vi "LB_FocusName_Tests.vi"(11 "error in":errorcluster) -> (15 "error out":errorcluster)   [LabVIEW 2016, in "DronaTest.lvlib"]
uses:
  DronaTest.lvlib
  APIs/Stimulus/ControlValue/SetValueAuto.vi
  APIs/Stimulus/ControlValue/Controls/Listbox/SetValueByItemName.vi
  APIs/Assert/AssertControlValue/Controls/Listbox/AssertValueByFocusName.vi
  APIs/Assert/AssertControlValue/Controls/Listbox/AssertValueByFocusIndex.vi
  <vilib>/addons/_JKI Toolkits/Caraya/classes/Assert/Assert Error.vi
  <vilib>/addons/_JKI Toolkits/Caraya/classes/Assert/Assert Equal Value_Variant.vi
  <vilib>/addons/_JKI Toolkits/Caraya/classes/Test/Test.lvclass
  Drona.lvlib
  <vilib>/SLL Toolkit/SLL Debug/SLL Debug.lvlib
  APIs/Stimulus/ControlValue/ControlValue.lvlib
  <vilib>/addons/_JKI Toolkits/Caraya/classes/Assert/Assert.lvclass
  APIs/Assert/AssertControlValue/Controls/Listbox/AssertListbox.lvlib
  APIs/Stimulus/ControlValue/Controls/Listbox/StimulusListbox.lvlib
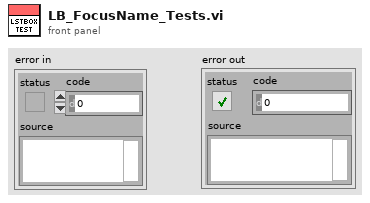
[diagram p1: front panel]
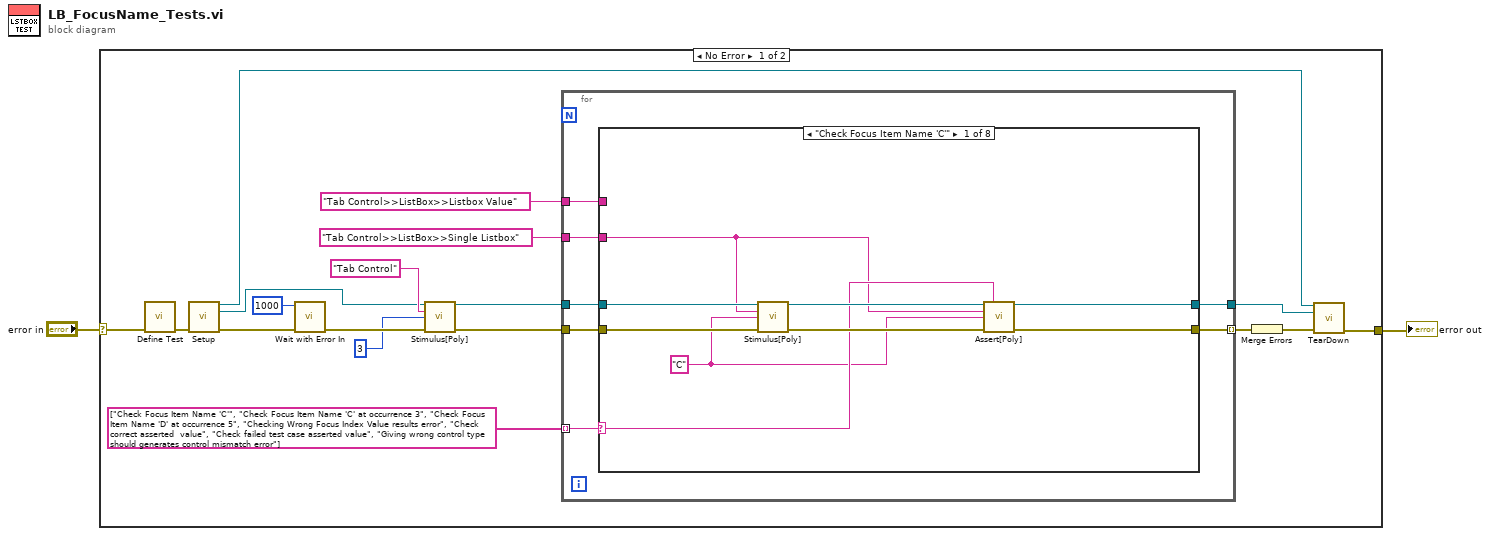
[diagram p0: block diagram]
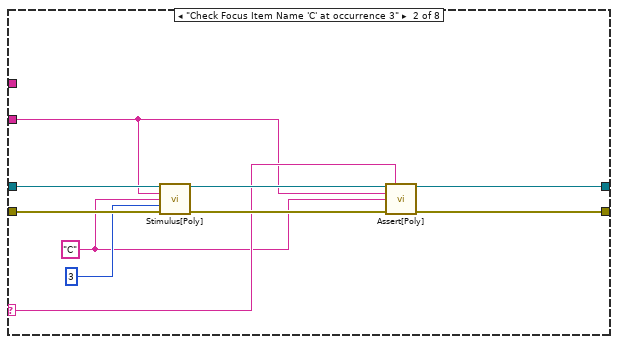
[diagram p2: hidden frame]
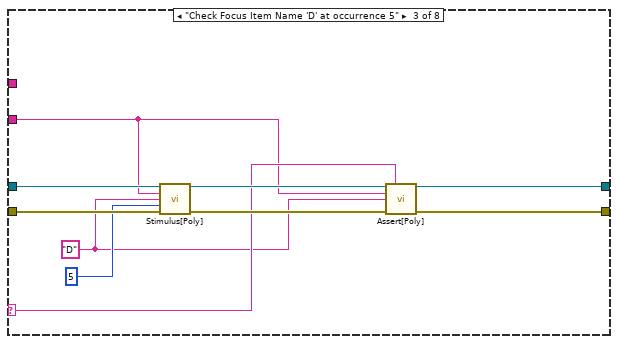
[diagram p3: hidden frame]
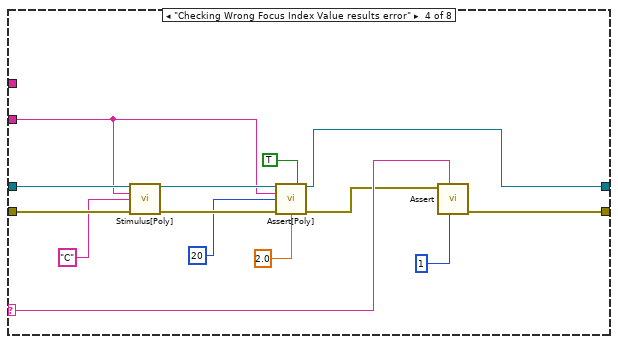
[diagram p4: hidden frame]
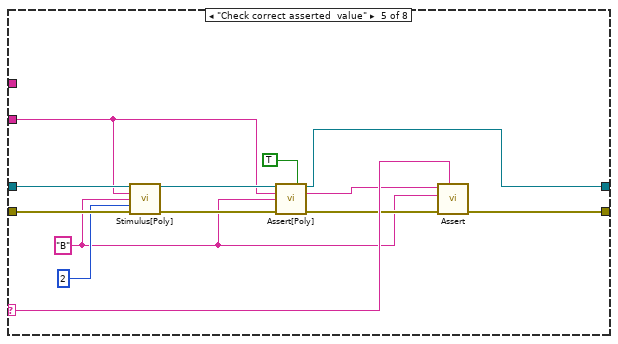
[diagram p5: hidden frame]
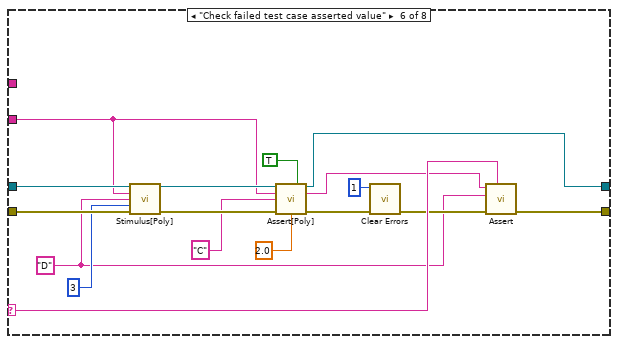
[diagram p6: hidden frame]
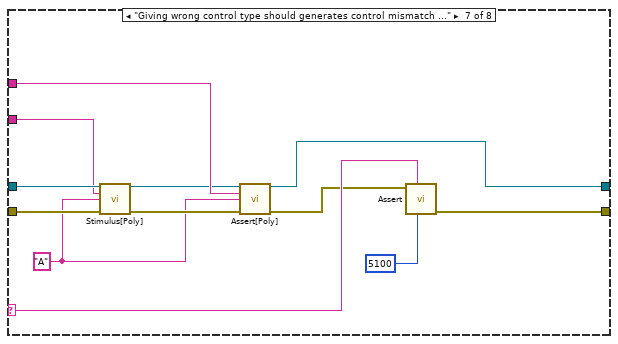
[diagram p7: hidden frame]
diagram:
  n1 = case shown="No Error" "error in" {
    selector: "error in" -> [w20 w115]
    tunnel: [w3 w115] -> w1
    frame No Error {
      n2 = call <vilib>:"Define Test.vi"("error in (no error)"=w20) -> ("error out"=w9:errorcluster)  [unwired: 9 in, 1 out]
      n3 = call "Setup.vi"("error in"=w9) -> ("Application Ref"=w5:refnum<vi>, "VI out"=w7:refnum<vi>, "error out"=w8:errorcluster)  [unwired: 12 in]
      n4 = call <vilib>:"Wait with Error In.vi"("error in (no error)"=w8, "milliseconds to wait"=u32 1000) -> ("error out"=w18:errorcluster)  [unwired: 9 in]
      n5 = call-poly "Stimulus[Poly].vi"("VI Reference In"=w7, "Control Path"="Tab Control", "Value (Signaling)"=3, "error in"=w18) -> ("VI Reference Out"=w14:refnum<vi>, "error out"=w17:errorcluster)  [unwired: 10 in]
      n6 = for {
        tunnel: w14 -> [w26]
        tunnel: "Tab Control>>ListBox>>Single Listbox" ("Control Path") -> [w25]
        tunnel: "Tab Control>>ListBox>>Listbox Value" ("Control Path") -> [w24]
        tunnel: string[] ["Check Focus Item Name 'C'", "Check Focus Item Name 'C' at occurrence 3", "Check Focus Item Name 'D' at occurrence 5", "Checking Wrong Focus Index Value results error", "Check correct asserted  value", "Check failed test case asserted value", "Giving wrong control type should generates control mismatch error"] -> [w22] mode=indexing
        tunnel: [w21] -> w4
        tunnel: w17 -> [w27]
        tunnel: [w23] -> w10 mode=indexing
        n7 = case shown="\"Check Focus Item Name 'C'\"" w22 {
          selector: w22 -> [w30 w40 w50 w69 w82 w99 w111 _]
          tunnel: w27 -> [w36 w46 w56 w67 w81 w98 w106 w114]
          tunnel: w26 -> [w35 w45 w55 w66 w80 w97 w104 w113]
          tunnel: w25 -> [w29 w39 w49 w63 w77 w94 w102 _]
          tunnel: w24 -> [_ _ _ _ _ _ w108 _]
          tunnel: [w32 w42 w52 w70 w83 w100 w112 w114] -> w23
          tunnel: [w31 w41 w51 w61 w76 w93 w107 w113] -> w21
          frame "Check Focus Item Name 'C'" {
            w28 = "C"
            n8 = call-poly "Stimulus[Poly].vi"("VI Reference In"=w35, "Control Path"=w29, "Item Name"=w28, "Error In"=w36) -> ("VI Reference Out"=w33:refnum<vi>, "Error Out"=w34:errorcluster)  [unwired: 10 in]
            n9 = call-poly "Assert[Poly].vi"("VI Reference In"=w33, "Test Label"=w30, "Control Path"=w29, "Item Name"=w28, "Error In"=w34) -> ("VI Reference Out"=w31:refnum<vi>, "Error Out"=w32:errorcluster)  [unwired: 8 in, 1 out]
          }
          frame "Check Focus Item Name 'C' at occurrence 3" {
            w37 = "C" ("Item Name")
            n10 = call-poly "Stimulus[Poly].vi"("VI Reference In"=w45, "Control Path"=w39, "Item Name"=w37, "Occurrence"=3 ("Item Index"), "Error In"=w46) -> ("VI Reference Out"=w43:refnum<vi>, "Error Out"=w44:errorcluster)  [unwired: 9 in]
            n11 = call-poly "Assert[Poly].vi"("VI Reference In"=w43, "Test Label"=w40, "Control Path"=w39, "Item Name"=w37, "Error In"=w44) -> ("VI Reference Out"=w41:refnum<vi>, "Error Out"=w42:errorcluster)  [unwired: 8 in, 1 out]
          }
          frame "Check Focus Item Name 'D' at occurrence 5" {
            w47 = "D" ("Item Name")
            n12 = call-poly "Stimulus[Poly].vi"("VI Reference In"=w55, "Control Path"=w49, "Item Name"=w47, "Occurrence"=5 ("Item Index"), "Error In"=w56) -> ("VI Reference Out"=w53:refnum<vi>, "Error Out"=w54:errorcluster)  [unwired: 9 in]
            n13 = call-poly "Assert[Poly].vi"("VI Reference In"=w53, "Test Label"=w50, "Control Path"=w49, "Item Name"=w47, "Error In"=w54) -> ("VI Reference Out"=w51:refnum<vi>, "Error Out"=w52:errorcluster)  [unwired: 8 in, 1 out]
          }
          frame "Checking Wrong Focus Index Value results error" {
            n14 = call-poly "Stimulus[Poly].vi"("VI Reference In"=w66, "Control Path"=w63, "Item Name"="C", "Error In"=w67) -> ("VI Reference Out"=w64:refnum<vi>, "Error Out"=w65:errorcluster)  [unwired: 10 in]
            n15 = call-poly "Assert[Poly].vi"("VI Reference In"=w64, "Assert Only? (F)"=TRUE, "Control Path"=w63, "Focus Index"=20 ("Item Index"), "Error In"=w65, "Timeout(5 sec)"=2.0) -> ("VI Reference Out"=w61:refnum<vi>, "Error Out"=w60:errorcluster)  [unwired: 7 in, 1 out]
            n16 = call-poly <vilib>:"Assert.vi"("error code (1)"=1, "Label"=w69, "Error?"=w60) -> ("error out"=w70:errorcluster)  [unwired: 7 in, 1 out]
          }
          frame "Check correct asserted  value" {
            w72 = "B" ("Item Name")
            n17 = call-poly "Stimulus[Poly].vi"("VI Reference In"=w80, "Control Path"=w77, "Item Name"=w72, "Occurrence"=2, "Error In"=w81) -> ("VI Reference Out"=w78:refnum<vi>, "Error Out"=w79:errorcluster)  [unwired: 9 in]
            n18 = call-poly "Assert[Poly].vi"("VI Reference In"=w78, "Assert Only? (F)"=TRUE, "Control Path"=w77, "Item Name"=w72, "Error In"=w79) -> ("VI Reference Out"=w76:refnum<vi>, "Asserted Value"=w74:string, "Error Out"=w75:errorcluster)  [unwired: 8 in]
            n19 = call-poly <vilib>:"Assert.vi"("Label"=w82, "error in (no error)"=w75, "Y"=w72, "X"=w74) -> ("error out"=w83:errorcluster)  [unwired: 6 in, 1 out]
          }
          frame "Check failed test case asserted value" {
            w84 = "D" ("Item Name")
            n20 = call-poly "Stimulus[Poly].vi"("VI Reference In"=w97, "Control Path"=w94, "Item Name"=w84, "Occurrence"=3, "Error In"=w98) -> ("VI Reference Out"=w95:refnum<vi>, "Error Out"=w96:errorcluster)  [unwired: 9 in]
            n21 = call-poly "Assert[Poly].vi"("VI Reference In"=w95, "Assert Only? (F)"=TRUE, "Control Path"=w94, "Item Name"="C", "Error In"=w96, "Timeout(5 sec)"=2.0) -> ("VI Reference Out"=w93:refnum<vi>, "Asserted Value"=w87:string, "Error Out"=w92:errorcluster)  [unwired: 7 in]
            n22 = call <vilib>:"Clear Errors.vi"("error in (no error)"=w92, "specific error code to clear (0: all)"=1) -> ("error out"=w89:errorcluster)  [unwired: 4 in, 1 out]
            n23 = call-poly <vilib>:"Assert.vi"("Label"=w99, "error in (no error)"=w89, "Y"=w84, "X"=w87) -> ("error out"=w100:errorcluster)  [unwired: 6 in, 1 out]
          }
          frame "Giving wrong control type should generates control mismatch error" {
            w101 = "A" ("Item Name")
            n24 = call-poly "Stimulus[Poly].vi"("VI Reference In"=w104, "Control Path"=w102, "Item Name"=w101, "Error In"=w106) -> ("VI Reference Out"=w103:refnum<vi>, "Error Out"=w105:errorcluster)  [unwired: 10 in]
            n25 = call-poly "Assert[Poly].vi"("VI Reference In"=w103, "Control Path"=w108, "Item Name"=w101, "Error In"=w105) -> ("VI Reference Out"=w107:refnum<vi>, "Error Out"=w109:errorcluster)  [unwired: 9 in, 1 out]
            n26 = call-poly <vilib>:"Assert.vi"("error code (1)"=5100, "Label"=w111, "Error?"=w109) -> ("error out"=w112:errorcluster)  [unwired: 7 in, 1 out]
          }
          frame Default {
          }
        }
      }
      n27 = Merge Errors(w10) -> (w6:errorcluster)
      n28 = call "TearDown.vi"("Application Ref"=w5, "VI in"=w4, "error in (no error)"=w6) -> ("error out"=w3:errorcluster)  [unwired: 12 in]
    }
    frame Error {
    }
  }
  "error out" <- w1
